vi "Decor.Listbox.vi"(7 "VI ref":refnum<vi>, 8 "error in (no error)":errorcluster, 10 "ctrl ref in":refnum<vi>, 11 "Material-Scheme in":refnum<class "Material-Scheme.lvclass">) -> (0 "error out":errorcluster)   [LabVIEW 2021, in "TSC Material Theme.lvlib" / "Material-Scheme.lvclass"]
uses:
  Material-Scheme.lvclass
  Material-Scheme.lvclass/Material-Scheme.ctl
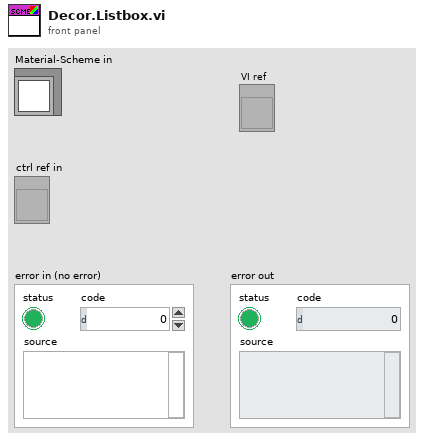
[diagram p1: front panel]
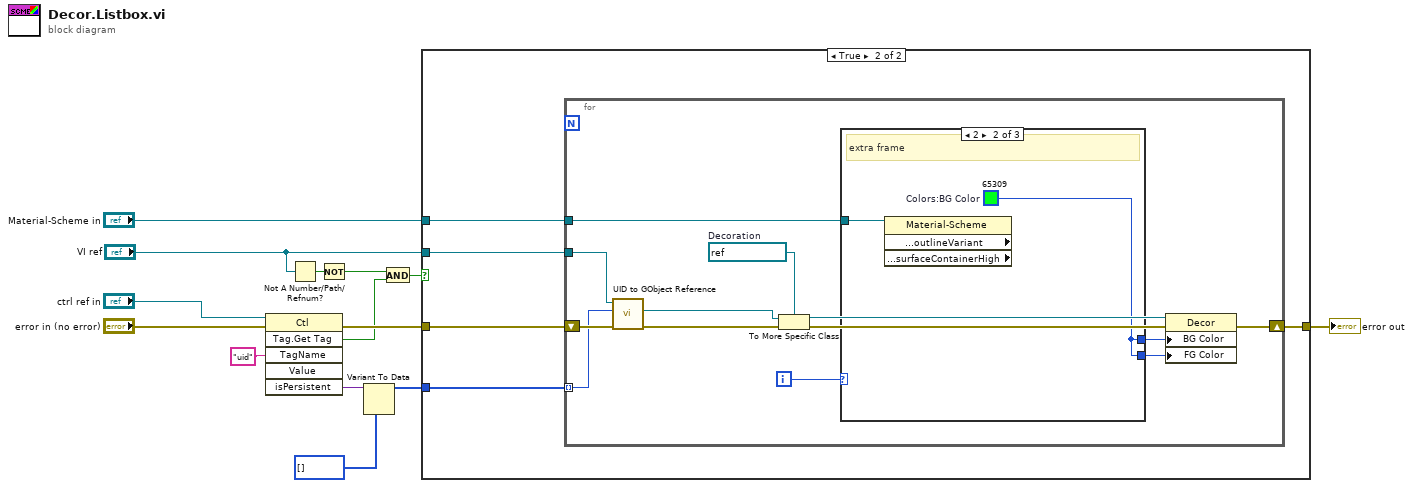
[diagram p0: block diagram]
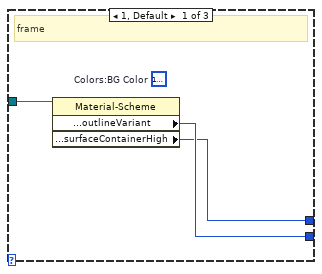
[diagram p3: hidden frame]
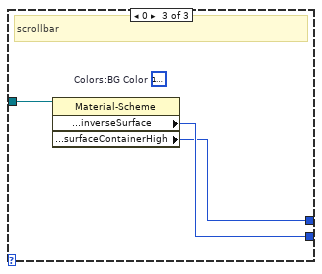
[diagram p4: hidden frame]
diagram:
  n1 = invoke class="Ctl" method="Tag.Get Tag"(reference="ctrl ref in", error in="error in (no error)", "TagName"="uid" ("Tag Name")) -> (error out=w9:errorcluster, "GetTag"=w5:bool, "isPersistent"=w13:variant)  [unwired: 3 in, 3 out]
  n2 = Not A Number/Path/Refnum?(number/path/refnum="VI ref") -> (NaN/Path/Refnum?=w3:bool)
  n3 = Not(x=w3) -> (.not. x?=w2:bool)
  n4 = Variant To Data(type=i32[] [], Variant=w13) -> (data=w7:i32[])  [unwired: 1 in, 1 out]
  n5 = And(x=w2, y=w5) -> (x .and. y?=w1:bool)
  n6 = case shown="True" w1 {
    tunnel: w9 -> [w15 w20]
    tunnel: [w15 w19] -> w8
    tunnel: "VI ref" -> [_ w18]
    tunnel: w7 -> [_ w17]
    tunnel: "Material-Scheme in" -> [_ w16]
    frame False {
    }
    frame True {
      n7 = for {
        tunnel: w18 -> [w31]
        shift-right: [w26] -> w19
        shift-left: w20 -> [w33]
        tunnel: w17 -> [w30] mode=indexing
        tunnel: w16 -> [w24]
        i -> [w21]
        w27 = refnum<vi> refnum  # Decoration
        n8 = call <vilib>:"UID to GObject Reference.vi"("error in (no error)"=w33, "UID"=w30, "Owning VI"=w31) -> ("error out"=w32:errorcluster, "GObject"=w28:refnum<vi>)  [unwired: 6 in, 1 out]
        n9 = To More Specific Class(target class=w27, reference=w28, error in=w32) -> (specific class reference=w25:refnum<vi>, error out=w29:errorcluster)
        n10 = case shown="2" w21 {
          tunnel: w24 -> [w36 w38 w41]
          tunnel: [w35 w37 w40] -> w23
          tunnel: [w34 w37 w39] -> w22
          frame 1, Default {
            (unwired) u32 16777216  # Colors:BG Color
            # "frame"
            n11 = property class="Material-Scheme"(reference=w36) -> ("data member access:Other:outlineVariant"=w35:u32, "data member access:Surface:surfaceContainerHigh"=w34:u32)  [unwired: 1 in, 2 out]
          }
          frame 2 {
            w37 = u32 65309  # Colors:BG Color
            # "extra frame"
            n12 = property class="Material-Scheme" props=["data member access:Other:outlineVariant", "data member access:Surface:surfaceContainerHigh"](reference=w38) -> ()  [unwired: 1 in, 4 out]
          }
          frame 0 {
            (unwired) u32 16777216  # Colors:BG Color
            # "scrollbar"
            n13 = property class="Material-Scheme"(reference=w41) -> ("data member access:Surface:inverseSurface"=w40:u32, "data member access:Surface:surfaceContainerHigh"=w39:u32)  [unwired: 1 in, 2 out]
          }
        }
        n14 = property class="Decor"(reference=w25, error in=w29, "BG Color"=w22, "FG Color"=w23) -> (error out=w26:errorcluster)  [unwired: 1 out]
      }
    }
  }
  "error out" <- w8
